vi "Cleanup When BD.vi"(8 "error in (no error)":errorcluster, 11 "VI in":refnum<vi>) -> (0 "error out":errorcluster, 3 "VI out":refnum<vi>)   [LabVIEW 2020, in "Mock Class Generator.lvclass"]
uses:
  Mock Class Generator.lvclass
  <vilib>/Utility/traverseref.llb/TRef TravTarget.ctl
  <vilib>/Utility/traverseref.llb/VI Scripting - Traverse.lvlib
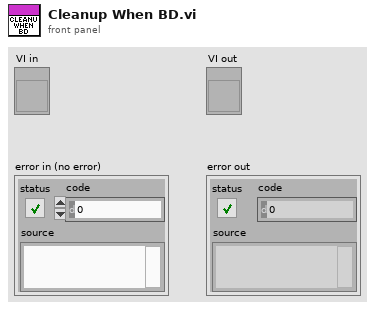
[diagram p1: front panel]
types:
  T1 = typedef "TRef TravTarget.ctl" = enum16{"FP", "BD", "Other"}
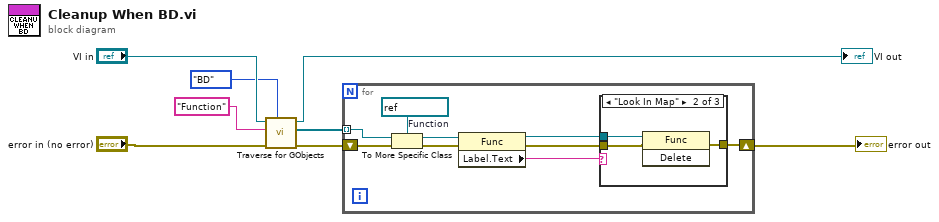
[diagram p0: block diagram]
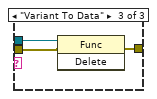
[diagram p3: hidden frame]
diagram:
  n1 = call <vilib>:"Traverse for GObjects.vi"("Traverse Target"=TRef_TravTarget."BD", "error in (no error)"="error in (no error)", "Class Name"="Function" ("name/order"), "VI Refnum"="VI in") -> ("error out"=w5:errorcluster, "References"=w4:refnum<vi>[], "dup VI Refnum"=→"VI out":refnum<vi>)  [unwired: 4 in, 1 out]
  n2 = for {
    tunnel: w4 -> [w11] mode=indexing
    shift-right: [w17] -> w2
    shift-left: w5 -> [w16]
    w9 = refnum<vi> refnum  # Function
    n3 = To More Specific Class(target class=w9, reference=w11, error in=w16) -> (specific class reference=w10:refnum<vi>, error out=w12:errorcluster)
    n4 = property class="Func"(reference=w10, error in=w12) -> (reference out=w14:refnum<vi>, error out=w15:errorcluster, "Label.Text"=w13:string)
    n5 = case shown="\"Look In Map\"" w13 {
      tunnel: [w18 w21 w24] -> w17
      tunnel: w15 -> [w18 w20 w23]
      tunnel: w14 -> [_ w19 w22]
      frame Default {
      }
      frame "Look In Map" {
        n6 = invoke class="Func" method="Delete"(reference=w19, error in=w20) -> (error out=w21:errorcluster)  [unwired: 1 in, 2 out]
      }
      frame "Variant To Data" {
        n7 = invoke class="Func" method="Delete"(reference=w22, error in=w23) -> (error out=w24:errorcluster)  [unwired: 1 in, 2 out]
      }
    }
  }
  "error out" <- w2
